vi "test prompt elicitation.vi"(8 "error in (no error)":errorcluster) -> (0 "error out":errorcluster, 3 "body":string)   [LabVIEW 2020, in "MCP Server tests.lvlib"]
doc: "Elicitation in prompts/get (MCP 2026-07-28). fake_prompt_ask_user calls Ask User.vi with the key context. A modern prompts/get from a client with the elicitation capability (id 72) is answered input_required with inputRequests.context and a requestState; the retry with inputResponses context accept {\"context\":\"the lab\"} and that requestState (id 721) is answered with a complete GetPromptResult whose message text contains the lab. The requests are sent with the LabVIEW HTTP Client directly."
uses:
  MCP Server tests.lvlib
  <vilib>/JDP Science/JSONtext/Next JSON Value.vi
  <vilib>/JDP Science/JSONtext/String Subset.vi
  <vilib>/JDP Science/JSONtext/support/Strip Quotes and Unescape.vi
  <vilib>/JDP Science/JSONtext/Parsing/Advance past next JSON Value (inlined COPY).vi
  <vilib>/JDP Science/JSONtext/support/Unescape JSON string.vi
  <vilib>/JDP Science/JSONtext/Parsing/Advance past whitespace.vi
  <vilib>/JDP Science/JSONtext/Parsing/Advance past String.vi
  <vilib>/JDP Science/JSONtext/Parsing/Advance past Number.vi
  <vilib>/JDP Science/JSONtext/Parsing/Advance past Line Ending.vi
  <vilib>/JDP Science/JSONtext/Parsing/Parse Full Path or Item Name.vi
  <vilib>/JDP Science/JSONtext/Parsing/Advance past Array.vi
  <vilib>/JDP Science/JSONtext/Parsing/Advance past Object.vi
  <vilib>/JDP Science/JSONtext/support/Error Cluster From Code.vi
  <vilib>/JDP Science/JSONtext/Offset/Find Item Locations by Path.vi
  <vilib>/JDP Science/JSONtext/Parsing/Advance past next JSON Value.vi
  <vilib>/addons/_JKI Toolkits/Caraya/classes/Test/Test.lvclass
  <vilib>/JDP Science/JSONtext/JSONtext.lvlib
  <vilib>/addons/_JKI Toolkits/Caraya/classes/Assert/Assert.lvclass
panel:
  out "lookup error":errorcluster
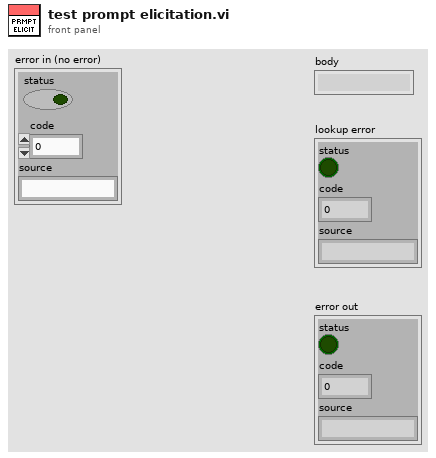
[diagram p1: front panel]
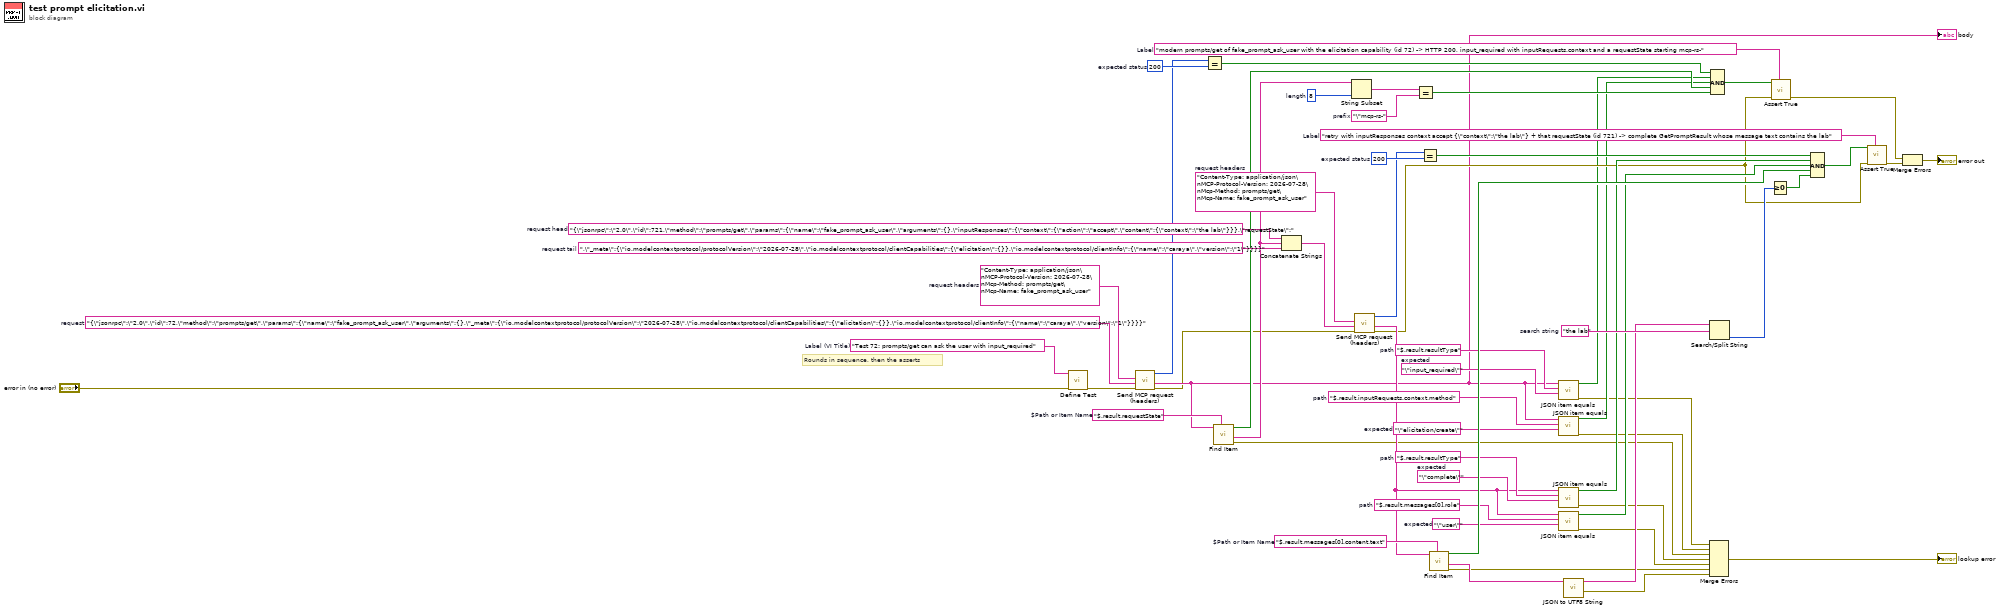
[diagram p0: block diagram]
diagram:
  w57 = "retry with inputResponses context accept {\"context\":\"the lab\"} + that requestState (id 721) -> complete GetPromptResult whose message text contains the lab"  # Label
  w54 = "modern prompts/get of fake_prompt_ask_user with the elicitation capability (id 72) -> HTTP 200, input_required with inputRequests.context and a requestState starting mcp-rs-"  # Label
  w50 = "the lab"  # search string
  w44 = "$.result.messages[0].content.text"  # $Path or Item Name
  w41 = "\"user\""  # expected
  w40 = "$.result.messages[0].role"  # path
  w37 = "\"complete\""  # expected
  w36 = "$.result.resultType"  # path
  w34 = 200  # expected status
  w30 = "Content-Type: application/json\nMCP-Protocol-Version: 2026-07-28\nMcp-Method: prompts/get\nMcp-Name: fake_prompt_ask_user"  # request headers
  w28 = ",\"_meta\":{\"io.modelcontextprotocol/protocolVersion\":\"2026-07-28\",\"io.modelcontextprotocol/clientCapabilities\":{\"elicitation\":{}},\"io.modelcontextprotocol/clientInfo\":{\"name\":\"caraya\",\"version\":\"1\"}}}}"  # request tail
  w27 = "{\"jsonrpc\":\"2.0\",\"id\":721,\"method\":\"prompts/get\",\"params\":{\"name\":\"fake_prompt_ask_user\",\"arguments\":{},\"inputResponses\":{\"context\":{\"action\":\"accept\",\"content\":{\"context\":\"the lab\"}}},\"requestState\":"  # request head
  w24 = 8  # length
  w23 = "\"mcp-rs-"  # prefix
  w19 = "$.result.requestState"  # $Path or Item Name
  w16 = "\"elicitation/create\""  # expected
  w15 = "$.result.inputRequests.context.method"  # path
  w12 = "\"input_required\""  # expected
  w11 = "$.result.resultType"  # path
  w9 = 200  # expected status
  w5 = "Content-Type: application/json\nMCP-Protocol-Version: 2026-07-28\nMcp-Method: prompts/get\nMcp-Name: fake_prompt_ask_user"  # request headers
  w4 = "{\"jsonrpc\":\"2.0\",\"id\":72,\"method\":\"prompts/get\",\"params\":{\"name\":\"fake_prompt_ask_user\",\"arguments\":{},\"_meta\":{\"io.modelcontextprotocol/protocolVersion\":\"2026-07-28\",\"io.modelcontextprotocol/clientCapabilities\":{\"elicitation\":{}},\"io.modelcontextprotocol/clientInfo\":{\"name\":\"caraya\",\"version\":\"1\"}}}}"  # request
  w2 = "Test 72: prompts/get can ask the user with input_required"  # Label (VI Title)
  # "Rounds in sequence, then the asserts"
  n1 = call <vilib>:"Define Test.vi"("error in (no error)"="error in (no error)", "Label (VI Title)"=w2) -> ("error out"=w3:errorcluster)  [unwired: 8 in, 1 out]
  n2 = call "Send MCP request (headers).vi"("error in (no error)"=w3, "request"=w4, "request headers"=w5) -> ("error out"=w6:errorcluster, "response"=w7:string, "status code"=w8:i32)  [unwired: 5 in, 1 out]
  "body" <- w7
  n3 = Equal?(x=w8, y=w9) -> (x = y?=w10:bool)
  n4 = call <vilib>:"Find Item.vi"("$Path or Item Name"=w19, "JSON"=w7) -> ("error out"=w20:errorcluster, "<JSON>"=w21:string, "Found"=w22:bool)  [unwired: 6 in, 1 out]
  n5 = Concatenate Strings(w27, w21, w28) -> (w29:string)
  n6 = String Subset(string=w21, length (rest)=w24) -> (substring=w25:string)  [unwired: 1 in]
  n7 = call "Send MCP request (headers).vi"("error in (no error)"=w6, "request"=w29, "request headers"=w30) -> ("error out"=w31:errorcluster, "response"=w32:string, "status code"=w33:i32)  [unwired: 5 in, 1 out]
  n8 = Equal?(x=w25, y=w23) -> (x = y?=w26:bool)
  n9 = Equal?(x=w33, y=w34) -> (x = y?=w35:bool)
  n10 = call <vilib>:"Find Item.vi"("$Path or Item Name"=w44, "JSON"=w32) -> ("error out"=w45:errorcluster, "<JSON>"=w46:string, "Found"=w47:bool)  [unwired: 6 in, 1 out]
  n11 = call "JSON item equals.vi"("expected"=w12, "path"=w11, "JSON"=w7) -> ("error out"=w13:errorcluster, "equal?"=w14:bool)  [unwired: 6 in, 1 out]
  n12 = call "JSON item equals.vi"("expected"=w16, "path"=w15, "JSON"=w7) -> ("error out"=w17:errorcluster, "equal?"=w18:bool)  [unwired: 6 in, 1 out]
  n13 = call "JSON item equals.vi"("expected"=w37, "path"=w36, "JSON"=w32) -> ("error out"=w38:errorcluster, "equal?"=w39:bool)  [unwired: 6 in, 1 out]
  n14 = call "JSON item equals.vi"("expected"=w41, "path"=w40, "JSON"=w32) -> ("error out"=w42:errorcluster, "equal?"=w43:bool)  [unwired: 6 in, 1 out]
  n15 = call <vilib>:"JSON to UTF8 String.vi"("JSON"=w46) -> ("error out"=w49:errorcluster, "<UTF8>String"=w48:string)  [unwired: 9 in]
  n16 = Merge Errors(w13, w17, w20, w38, w42, w45, w49) -> (→"lookup error":errorcluster)
  n17 = Search/Split String(string=w48, search string/char (-)=w50) -> (offset of match=w51:i32)  [unwired: 1 in, 2 out]
  n18 = Compound Arithmetic op=AND(w10, w14, w18, w22, w26) -> (w53:bool)
  n19 = Greater Or Equal To 0?(x=w51) -> (x >= 0?=w52:bool)
  n20 = call <vilib>:"Assert True.vi"("Label"=w54, "error in (no error)"=w31, "True?"=w53) -> ("error out"=w55:errorcluster)  [unwired: 7 in, 1 out]
  n21 = Compound Arithmetic op=AND(w35, w39, w43, w47, w52) -> (w56:bool)
  n22 = call <vilib>:"Assert True.vi"("Label"=w57, "error in (no error)"=w31, "True?"=w56) -> ("error out"=w58:errorcluster)  [unwired: 7 in, 1 out]
  n23 = Merge Errors(w55, w58) -> (→"error out":errorcluster)
